vi "Pigeon2 Field Centric.vi"(10 "Field Centric Velocities":T1) -> (3 "Robot Centric Velocities":T1)   [LabVIEW 2023]
uses:
  <vilib>/MRC/MrcLib.lvlib
  <vilib>/MRC/MrcLib/VIs/IMU/IMU Get Yaw Flat.vi
  Type Definitions/Data/Robot Velocities.ctl
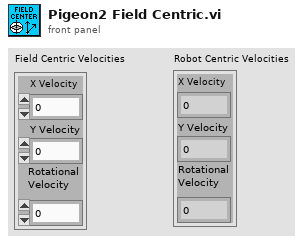
[diagram p1: front panel]
types:
  T1 = typedef "Robot Velocities.ctl" = cluster{"X Velocity":dbl, "Y Velocity":dbl, "Rotational \nVelocity":dbl}
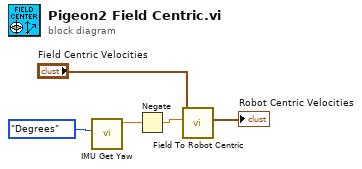
[diagram p0: block diagram]
diagram:
  n1 = call-poly <vilib>:"IMU Get Yaw.vi"("Units"=enum16{"Radians", "Degrees"}."Degrees") -> ("yaw"=w2:dbl)  [unwired: 8 in, 2 out]
  n2 = Negate(x=w2) -> (-x=w1:dbl)
  n3 = call "Field To Robot Centric.vi"("IMU Value (offset)"=w1, "Field Centric Velocities"="Field Centric Velocities") -> ("Robot Centric Velocities"=→"Robot Centric Velocities":T1)  [unwired: 8 in, 1 out]
